vi "GDM-9052 Read DC Voltage.vi"() -> ()   [LabVIEW 2021, in "GDM-9052.lvlib"]
uses:
  GDM-9052.lvlib
panel:
  in  "Manual Range":dbl format="%#.9e"
  in  "Configure RS232 Baud Rate":u32(ring)=115200 items=["9600"=9600, "19200"=19200, "38400"=38400, "57600"=57600, "115200"=115200]
  out "error out":errorcluster
  out "Measure Value":string
  in  "Stop":bool
  out "Boolean":bool
  in  "Detector Rate":u8(ring) items=["SLOW", "MID", "FAST"]
  in  "Enable Auto Range":bool=TRUE
  out "ID Return String":string
  in  "VISA resource name":refnum<visa-resource-name>
  # "GDM-9052 Read DC Voltage"
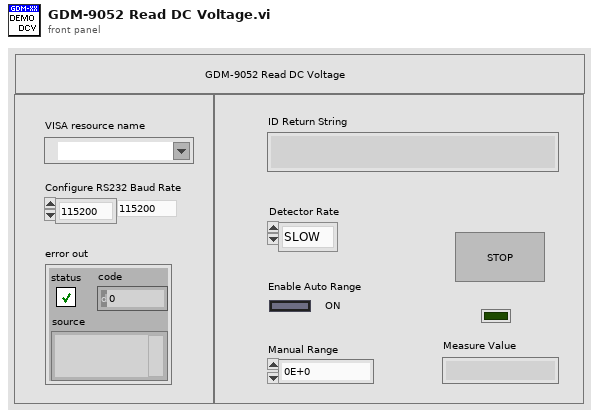
[diagram p1: front panel]
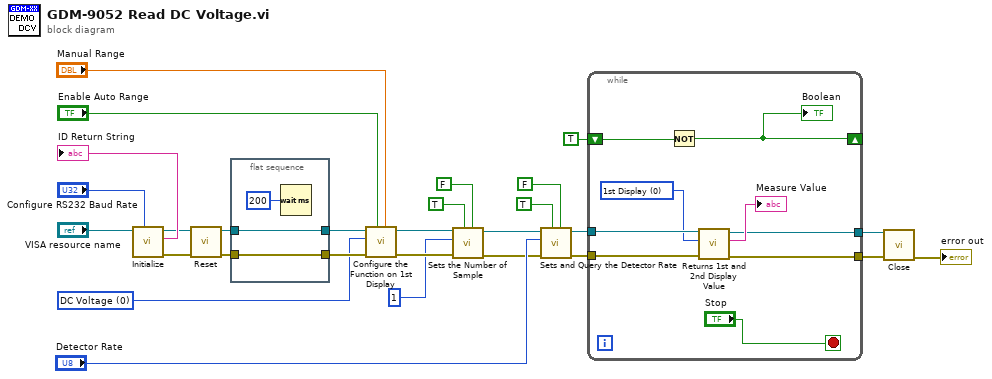
[diagram p0: block diagram]
diagram:
  w2 = u8 0 items=["DC Voltage", "AC Voltage", "DC Current", "AC Current", "2-Wire Resistance", "4-Wire Resistance", "Frequency", "Period", "Continuity", "Diode", "Temperature", "Capacitance"] ("Function")
  n1 = call "Initialize.vi"("Configure RS232 Baud Rate"="Configure RS232 Baud Rate", "VISA resource name"="VISA resource name") -> ("error out"=w16:errorcluster, "ID Return String"=→"ID Return String":string, "VISA resource name out"=w17:refnum<visa-resource-name>)  [unwired: 6 in, 1 out]
  n2 = call "Reset.vi"("error in (no error)"=w16, "VISA resource name"=w17) -> ("error out"=w12:errorcluster, "VISA resource name out"=w14:refnum<visa-resource-name>)  [unwired: 8 in]
  n3 = flat-sequence {
    tunnel: w14 -> [w31]
    tunnel: [w31] -> w13
    tunnel: w12 -> [w30]
    tunnel: [w30] -> w11
    frame #0 {
      n4 = Wait (ms)(milliseconds to wait=u32 200) -> ()  [unwired: 1 out]
    }
  }
  n5 = call "Configure the Function on 1st Display .vi"("Manual Range"="Manual Range", "Enable Auto Range"="Enable Auto Range", "error in"=w11, "Function"=w2, "VISA resource name"=w13) -> ("error out"=w9:errorcluster, "VISA resource name out"=w10:refnum<visa-resource-name>)  [unwired: 5 in]
  n6 = call "Sets the Number of Sample.vi"("Enable to Query"=FALSE, "Enable to Sets"=TRUE, "error in"=w9, "Number of Sample"=u16 1, "VISA resource name"=w10) -> ("error out"=w7:errorcluster, "VISA resource name out"=w8:refnum<visa-resource-name>)  [unwired: 4 in, 1 out]
  n7 = call "Sets and Query the Detector Rate.vi"("Enable to Query"=FALSE, "Enable to Sets"=TRUE, "error in"=w7, "Detector Rate"="Detector Rate", "VISA resource name"=w8) -> ("error out"=w21:errorcluster, "VISA resource name out"=w22:refnum<visa-resource-name>)  [unwired: 4 in, 1 out]
  n8 = while {
    tunnel: w22 -> [w40]
    tunnel: w21 -> [w39]
    tunnel: [w35] -> w20
    tunnel: [w34] -> w19
    shift-right: [w32] -> _
    shift-left: TRUE -> [w33]
    stop <- "Stop" stop-if-true
    w38 = u16 0 items=["1st Display", "2nd Display", "1st & 2nd Display"] ("Sets to Display")
    n9 = Not(x=w33) -> (.not. x?=w32:bool)
    "Boolean" <- w32
    n10 = call "Returns 1st and 2nd Display Value.vi"("error in"=w39, "Sets to Display"=w38, "VISA resource name"=w40) -> ("error out"=w34:errorcluster, "Return the Value"=→"Measure Value":string, "VISA resource name out"=w35:refnum<visa-resource-name>)  [unwired: 6 in]
  }
  n11 = call "Close.vi"("error in (no error)"=w19, "VISA resource name"=w20) -> ("error out"=→"error out":errorcluster)  [unwired: 9 in]
